vi "AT1B_Radar.vi"() -> ()   [LabVIEW 2026]
doc: "Virtuelle 4-20-mA-Kette mit eigenem Trend; keine HART- oder DTM-Verbindung. Sensor und Auswertung getrennt abgleichen. Weitere Einstellungen unterhalb der Aufnahme.\nGeometrie und liegender Zylinder sind Beispiele."
panel:
  out "Bewegungsparameter gueltig":bool=TRUE
  out "Grafikfehlercode":i32
  out "Stromverlauf [mA] - 20 ms je Punkt":dbl(graph)
  out "CSV-Fehlercode":i32
  out "Ungespeicherte Daten":bool
  out "Zeilen aufgenommen":i32
  out "Aufnahmestatus":string
  in  "Pruefstand beenden":bool
  in  "Neue CSV-Datei":path
  in  "CSV speichern":bool
  in  "Ungespeicherte Aufnahme verwerfen erlauben":bool
  in  "Neue Aufnahme":bool
  in  "Aufnahme eingeschaltet":bool
  out "Abgleichfehler (0 / 1 / 2)":dbl
  out "Signalzustand":string="Mit Ausfuehren / Strg+R starten."
  out "Messung angehalten - Anzeige historisch":bool
  out "Relais 2":bool
  out "Skalenwert":dbl=nan
  out "Auswertung linearisiert [%]":dbl=nan
  out "Auswertung [%]":dbl=nan
  out "Strom [mA]":dbl=nan
  out "Sensor linearisiert [%]":dbl=nan
  out "Sensor [%]":dbl=nan
  out "Distanz [m]":dbl=nan
  in  "Messung eingeschaltet":bool=TRUE
  in  "Auswertung uebernehmen":bool
  in  "Relais 2 Betriebsart":enum16{"Aus", "Fenster ein", "Fenster aus"}(ring)
  in  "Relais 2 Obergrenze [%]":dbl
  in  "Relais 2 Untergrenze [%]":dbl
  in  "Skalenwert bei 100 %":dbl
  in  "Skalenwert bei 0 %":dbl
  in  "Auswertung Linearisierung":enum16{"Linear", "Zylinder liegend - Beispiel"}(ring)
  in  "Auswertung Strom bei 100 % [mA]":dbl=20.0
  in  "Auswertung Strom bei 0 % [mA]":dbl=4.0
  in  "Sensorabgleich uebernehmen":bool
  in  "Sensor-Linearisierung":enum16{"Linear", "Zylinder liegend - Beispiel"}(ring)
  in  "Sensordistanz bei 100 % [m]":dbl
  in  "Sensordistanz bei 0 % [m]":dbl
  in  "Daempfung [s]":dbl
  in  "Messoffset [m] - Beispiel":dbl
  in  "Sensorhoehe ueber Boden [m] - Beispiel":dbl=1.5
  in  "Echo vorhanden":bool=TRUE
  in  "Geraete eingeschaltet":bool=TRUE
  out "Abgeschlossene Fahrten":dbl
  out "Fahrt aktiv":bool
  out "Position aktuell":dbl
  in  "Bewegung pausieren":bool
  in  "Bewegung stoppen":bool
  in  "Ablauf starten":bool
  in  "Schrittweite":dbl=0.01
  in  "Fahrtart":enum16{"Pendeln", "Schritte", "Einfachfahrt"}(ring)
  in  "Wiederholungen":dbl=1.0
  in  "Haltezeit [s]":dbl=0.5
  in  "Tempo pro Sekunde":dbl=0.05
  in  "Endposition":dbl=1.2
  in  "Startposition":dbl
  in  "Position setzen":bool
  in  "Handposition":dbl=0.3
  out "Kurzhilfe":string="Virtuelle 4-20-mA-Kette mit eigenem Trend; keine HART- oder DTM-Verbindung. Sensor und Auswertung getrennt abgleichen. Weitere Einstellungen unterhalb der Aufnahme.\nGeometrie und liegender Zylinder sind Beispiele."
  out "Pruefstand":string="AT-1B / VEGAPULS C22 und VEGAMET 391 - Fuellhoehe in m"
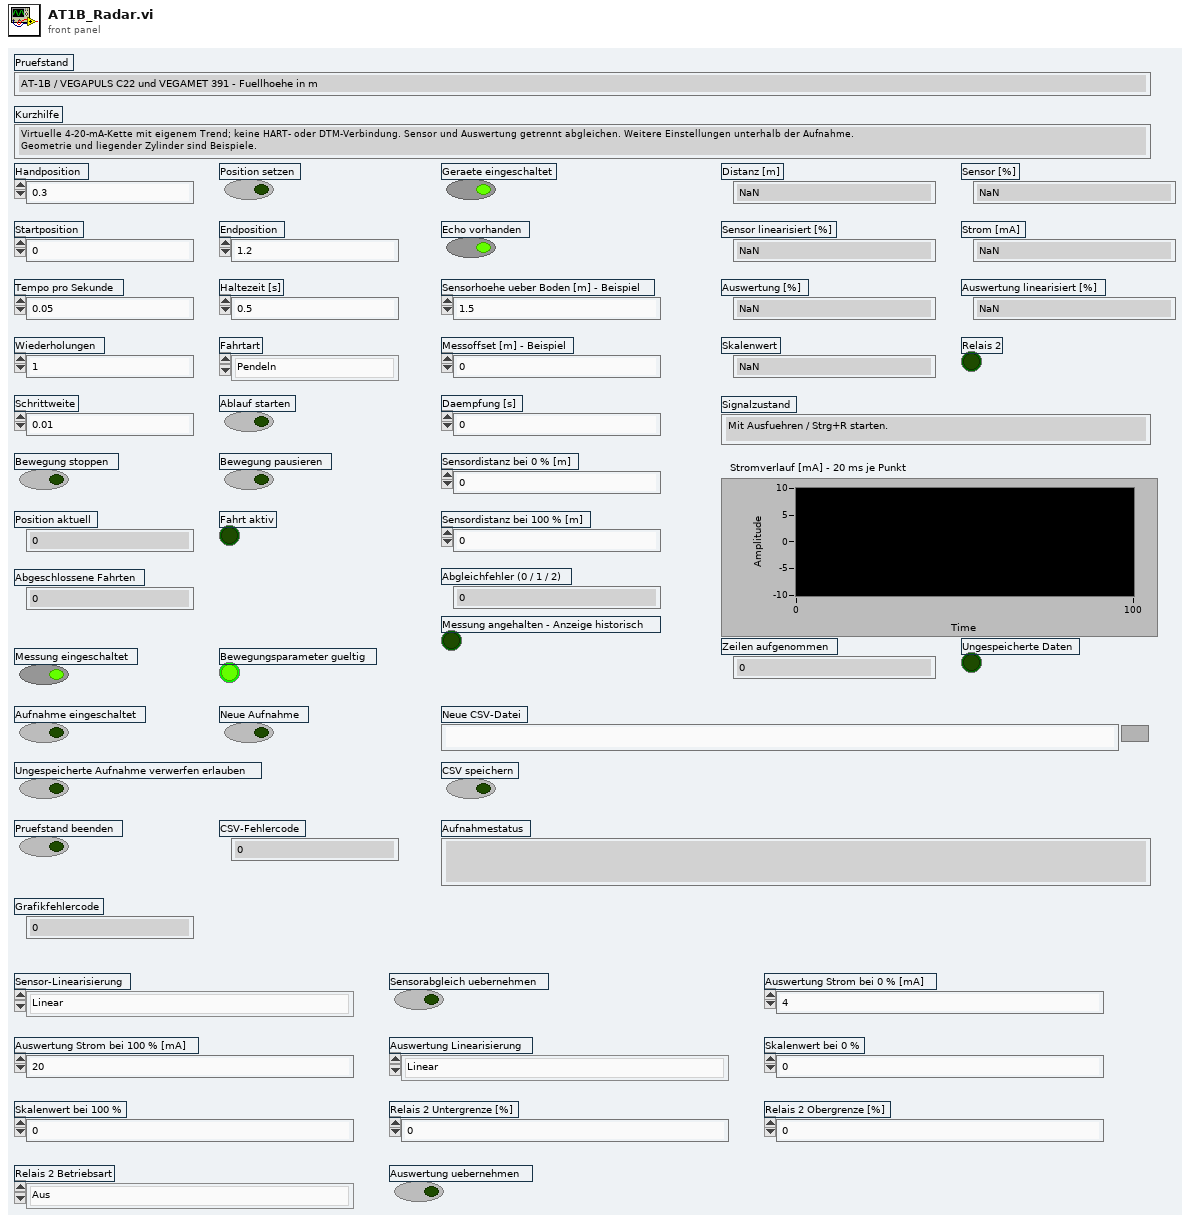
[diagram p1: front panel]
types:
  T1 = cluster{"record":bool, "clear":bool, "limit":i32, "header":string, "source":string}
diagram:
  n1 = while {
    shift-right: [w27] -> _
    shift-left: dbl[] [0.0, 0.0, 0.0, 0.0, 0.0, 0.0, 0.0, 0.0, 0.0, 0.0, 0.0, 0.0] -> [w26]
    shift-right: [w87] -> _
    shift-left: dbl[] [0.0, 0.0, 0.0, 0.0, 0.0, 0.0, 0.0, 0.0, 0.0, 0.0, 0.0, 0.0, 0.0, 0.0, 0.0, 0.0, 0.0, 0.0, 0.0, 0.0] -> [w86]
    shift-right: [w92] -> _
    shift-left: dbl[] [nan, nan, nan, nan, nan, nan, nan, nan] -> [w91]
    shift-right: [w164] -> _
    shift-left: cluster{"text":string, "count":i32} {"text"="Quelle;Zeit_s;Fuellhoehe_m;Distanz_m;Sensor_pct;Sensor_linear_pct;Strom_mA;Auswertung_pct;Auswertung_linear_pct;Skalenwert;Relais2;Qualitaet;Parameterfehler;Eingang_dt_s;Eingang_sensor_plane_above_bottom_m_example;Eingang_fill_height_m;Eingang_echo;Eingang_power;Eingang_offset_m_example;Eingang_damping_s;Eingang_sensor_distance_at_0pct_m;Eingang_sensor_distance_at_100pct_m;Eingang_sensor_linearization_0_linear_1_horizontal_cylinder;Eingang_sensor_apply_pressed;Eingang_controller_current_at_0pct_mA;Eingang_controller_current_at_100pct_mA;Eingang_controller_linearization_0_linear_1_horizontal_cylinder;Eingang_scaled_0pct;Eingang_scaled_100pct;Eingang_relay_lower_pct;Eingang_relay_upper_pct;Eingang_relay_mode_0_off_1_window_on_2_window_off;Eingang_controller_apply_pressed\r\n", "count"=0} -> [w163]
    shift-right: [w166] -> _
    shift-left: 0 -> [w165]
    shift-right: [w227] -> _
    shift-left: errorcluster {"status"=FALSE, "code"=0, "source"=""} -> [w226]
    i -> [w7]
    stop <- w243 stop-if-true
    w10 = FALSE
    (unwired) 1.0
    w9 = 0.0
    w8 = 0.02
    # "Virtueller Pruefstand - 20 ms Modellschritt"
    n2 = case shown="True" "Position setzen" {
      frame False {
      }
      frame True {
        n3 = property on="Position setzen" class="Bool. (strikt)"("Value"=FALSE) -> ()  [unwired: 2 in, 2 out]
      }
    }
    n4 = case shown="True" "Ablauf starten" {
      frame False {
      }
      frame True {
        n5 = property on="Ablauf starten" class="Bool. (strikt)"("Value"=FALSE) -> ()  [unwired: 2 in, 2 out]
      }
    }
    n6 = case shown="True" "Bewegung stoppen" {
      frame False {
      }
      frame True {
        n7 = property on="Bewegung stoppen" class="Bool. (strikt)"("Value"=FALSE) -> ()  [unwired: 2 in, 2 out]
      }
    }
    n8 = case shown="True" "Sensorabgleich uebernehmen" {
      frame False {
      }
      frame True {
        n9 = property on="Sensorabgleich uebernehmen" class="Bool. (strikt)"("Value"=FALSE) -> ()  [unwired: 2 in, 2 out]
      }
    }
    n10 = case shown="True" "Auswertung uebernehmen" {
      frame False {
      }
      frame True {
        n11 = property on="Auswertung uebernehmen" class="Bool. (strikt)"("Value"=FALSE) -> ()  [unwired: 2 in, 2 out]
      }
    }
    n12 = case shown="True" "Neue Aufnahme" {
      frame False {
      }
      frame True {
        n13 = property on="Neue Aufnahme" class="Bool. (strikt)"("Value"=FALSE) -> ()  [unwired: 2 in, 2 out]
      }
    }
    n14 = case shown="True" "CSV speichern" {
      frame False {
      }
      frame True {
        n15 = property on="CSV speichern" class="Bool. (strikt)"("Value"=FALSE) -> ()  [unwired: 2 in, 2 out]
      }
    }
    n16 = case shown="True" "Pruefstand beenden" {
      frame False {
      }
      frame True {
        n17 = property on="Pruefstand beenden" class="Bool. (strikt)"("Value"=FALSE) -> ()  [unwired: 2 in, 2 out]
      }
    }
    n18 = Wait (ms)(milliseconds to wait=u32 20) -> ()  [unwired: 1 out]
    n19 = Select(t=1.0, s="Ablauf starten", f=0.0) -> (s? t:f=w30:dbl)
    n20 = property on="Stromverlauf [mA] - 20 ms je Punkt" class="SVDiagr (strikt)"("Legend:Visible"=w10, "Palette:Visible"=w10, "Scale Legend:Visible"=w10, "Position"=cluster{"Left":i32, "Top":i32} {"Left"=735, "Top"=420}, "Plot Area:Size"=cluster{"Width":u32, "Height":u32} {"Width"=340, "Height"=110}) -> (error out=w261:errorcluster)  [unwired: 2 in, 1 out]
    n21 = Select(t=1.0, s="Bewegung pausieren", f=0.0) -> (s? t:f=w33:dbl)
    n22 = Select(t=1.0, s="Position setzen", f=0.0) -> (s? t:f=w36:dbl)
    n23 = Select(t=1.0, s="Bewegung stoppen", f=0.0) -> (s? t:f=w39:dbl)
    n24 = Select(t=1.0, s="Echo vorhanden", f=0.0) -> (s? t:f=w76:dbl)
    n25 = Select(t=1.0, s="Geraete eingeschaltet", f=0.0) -> (s? t:f=w79:dbl)
    n26 = Select(t=1.0, s="Sensorabgleich uebernehmen", f=0.0) -> (s? t:f=w82:dbl)
    n27 = Select(t=1.0, s="Auswertung uebernehmen", f=0.0) -> (s? t:f=w85:dbl)
    n28 = Not(x="Messung eingeschaltet") -> (.not. x?=→"Messung angehalten - Anzeige historisch":bool)
    n29 = And(x="Aufnahme eingeschaltet", y="Messung eingeschaltet") -> (x .and. y?=w175:bool)
    n30 = Unbundle By Name(w163) -> ("count"=w167:i32)  [unwired: 1 out]
    n31 = Equal?(x=w7, y=w9) -> ()  [unwired: 1 out]
    n32 = Quotient & Remainder(x=w7, y=5) -> (x-y*floor(x/y)=w173:i32)  [unwired: 1 out]
    n33 = Build Array(w8, "Startposition", "Endposition", "Tempo pro Sekunde", "Haltezeit [s]", "Wiederholungen", w30, w33, w36, "Handposition", "Fahrtart", "Schrittweite", w39) -> (w40:dbl[])
    n34 = Unbundle By Name(w261) -> ("code"=→"Grafikfehlercode":i32)
    n35 = Greater?(x=w167, y=w165) -> (0:w168:bool)
    n36 = Equal?(x=w173, y=w9) -> (x = y?=w174:bool)
    n37 = call "Trajektorie.vi"("StateIn"=w26, "Parameters"=w40) -> ("Values"=w41:dbl[], "StateOut"=w27:dbl[])  [unwired: 8 in]
    n38 = Not(x=w168) -> (.not. x?=w169:bool)
    n39 = And(x=w175, y=w174) -> (x .and. y?=w176:bool)
    n40 = Index Array(array=w41, index=0) -> (element=w43:dbl)
    "Position aktuell" <- w43
    n41 = Index Array(array=w41, index=3) -> (element=w45:dbl)
    n42 = Index Array(array=w41, index=4) -> (element=w47:dbl)
    n43 = Index Array(array=w41, index=1) -> (element=w51:dbl)
    n44 = Index Array(array=w41, index=2) -> (element=→"Abgeschlossene Fahrten":dbl)
    n45 = Or(x=w169, y="Ungespeicherte Aufnahme verwerfen erlauben") -> (x .or. y?=w170:bool)
    n46 = Greater?(x=w47, y=0.0) -> (0:→"Bewegungsparameter gueltig":bool)
    n47 = Greater?(x=w51, y=0.0) -> (0:→"Fahrt aktiv":bool)
    n48 = Build Array(w8, "Sensorhoehe ueber Boden [m] - Beispiel", w43, w76, w79, "Messoffset [m] - Beispiel", "Daempfung [s]", "Sensordistanz bei 0 % [m]", "Sensordistanz bei 100 % [m]", "Sensor-Linearisierung", w82, "Auswertung Strom bei 0 % [mA]", "Auswertung Strom bei 100 % [mA]", "Auswertung Linearisierung", "Skalenwert bei 0 %", "Skalenwert bei 100 %", "Relais 2 Untergrenze [%]", "Relais 2 Obergrenze [%]", "Relais 2 Betriebsart", w85) -> (w88:dbl[])
    n49 = And(x="Neue Aufnahme", y=w170) -> (x .and. y?=w171:bool)
    n50 = Not(x=w170) -> (.not. x?=w244:bool)
    n51 = call "Radar_Schritt.vi"("StateIn"=w86, "Parameters"=w88) -> ("Values"=w89:dbl[], "StateOut"=w87:dbl[])  [unwired: 8 in]
    n52 = Index Array(array=w88, index=0) -> (element=w183:dbl)
    n53 = Index Array(array=w88, index=1) -> (element=w185:dbl)
    n54 = Index Array(array=w88, index=2) -> (element=w187:dbl)
    n55 = Index Array(array=w88, index=3) -> (element=w189:dbl)
    n56 = Index Array(array=w88, index=4) -> (element=w191:dbl)
    n57 = Index Array(array=w88, index=5) -> (element=w193:dbl)
    n58 = Index Array(array=w88, index=6) -> (element=w195:dbl)
    n59 = Index Array(array=w88, index=7) -> (element=w197:dbl)
    n60 = Index Array(array=w88, index=8) -> (element=w199:dbl)
    n61 = Index Array(array=w88, index=9) -> (element=w201:dbl)
    n62 = Index Array(array=w88, index=10) -> (element=w203:dbl)
    n63 = Index Array(array=w88, index=11) -> (element=w205:dbl)
    n64 = Index Array(array=w88, index=12) -> (element=w207:dbl)
    n65 = Index Array(array=w88, index=13) -> (element=w209:dbl)
    n66 = Index Array(array=w88, index=14) -> (element=w211:dbl)
    n67 = Index Array(array=w88, index=15) -> (element=w213:dbl)
    n68 = Index Array(array=w88, index=16) -> (element=w215:dbl)
    n69 = Index Array(array=w88, index=17) -> (element=w217:dbl)
    n70 = Index Array(array=w88, index=18) -> (element=w219:dbl)
    n71 = Index Array(array=w88, index=19) -> (element=w221:dbl)
    n72 = Bundle By Name(cluster=T1 {"record"=FALSE, "clear"=FALSE, "limit"=10000, "header"="", "source"=""}, "record"=w176, "clear"=w171, "limit"=10000, "header"="Quelle;Zeit_s;Fuellhoehe_m;Distanz_m;Sensor_pct;Sensor_linear_pct;Strom_mA;Auswertung_pct;Auswertung_linear_pct;Skalenwert;Relais2;Qualitaet;Parameterfehler;Eingang_dt_s;Eingang_sensor_plane_above_bottom_m_example;Eingang_fill_height_m;Eingang_echo;Eingang_power;Eingang_offset_m_example;Eingang_damping_s;Eingang_sensor_distance_at_0pct_m;Eingang_sensor_distance_at_100pct_m;Eingang_sensor_linearization_0_linear_1_horizontal_cylinder;Eingang_sensor_apply_pressed;Eingang_controller_current_at_0pct_mA;Eingang_controller_current_at_100pct_mA;Eingang_controller_linearization_0_linear_1_horizontal_cylinder;Eingang_scaled_0pct;Eingang_scaled_100pct;Eingang_relay_lower_pct;Eingang_relay_upper_pct;Eingang_relay_mode_0_off_1_window_on_2_window_off;Eingang_controller_apply_pressed\r\n", "source"="AT1B_Radar;") -> (w181:T1)
    n73 = Select(t=errorcluster {"status"=FALSE, "code"=0, "source"=""}, s=w171, f=w226) -> (s? t:f=w232:errorcluster)
    n74 = Select(t=0, s=w171, f=w165) -> (s? t:f=w239:i32)
    n75 = And(x="Neue Aufnahme", y=w244) -> (x .and. y?=w245:bool)
    n76 = Select(t=w89, s="Messung eingeschaltet", f=w91) -> (s? t:f=w92:dbl[])
    n77 = Index Array(array=w89, index=8) -> (element=w108:dbl)
    n78 = Index Array(array=w89, index=9) -> (element=w113:dbl)
    n79 = Index Array(array=w89, index=10) -> (element=→"Abgleichfehler (0 / 1 / 2)":dbl)
    n80 = Index Array(array=w89, index=0) -> (element=w138:dbl)
    n81 = Index Array(array=w89, index=1) -> (element=w140:dbl)
    n82 = Index Array(array=w89, index=2) -> (element=w142:dbl)
    n83 = Index Array(array=w89, index=3) -> (element=w144:dbl)
    n84 = Index Array(array=w89, index=4) -> (element=w146:dbl)
    n85 = Index Array(array=w89, index=5) -> (element=w148:dbl)
    n86 = Index Array(array=w89, index=6) -> (element=w150:dbl)
    n87 = Index Array(array=w89, index=8) -> (element=w152:dbl)
    n88 = Index Array(array=w89, index=9) -> (element=w154:dbl)
    n89 = Index Array(array=w89, index=10) -> (element=w156:dbl)
    n90 = Index Array(array=w92, index=0) -> (element=→"Distanz [m]":dbl)
    n91 = Index Array(array=w92, index=1) -> (element=→"Sensor [%]":dbl)
    n92 = Index Array(array=w92, index=2) -> (element=→"Sensor linearisiert [%]":dbl)
    n93 = Index Array(array=w92, index=3) -> (element=→"Strom [mA]":dbl)
    n94 = Index Array(array=w92, index=4) -> (element=→"Auswertung [%]":dbl)
    n95 = Index Array(array=w92, index=5) -> (element=→"Auswertung linearisiert [%]":dbl)
    n96 = Index Array(array=w92, index=6) -> (element=→"Skalenwert":dbl)
    n97 = Greater?(x=w108, y=0.0) -> (0:→"Relais 2":bool)
    n98 = Equal?(x=w113, y=0.0) -> (x = y?=w116:bool)
    n99 = Equal?(x=w113, y=1.0) -> (x = y?=w120:bool)
    n100 = Equal?(x=w113, y=2.0) -> (x = y?=w124:bool)
    n101 = Equal?(x=w113, y=3.0) -> (x = y?=w128:bool)
    n102 = Equal?(x=w113, y=4.0) -> (x = y?=w132:bool)
    n103 = Build Array(w45, w43, w138, w140, w142, w144, w146, w148, w150, w152, w154, w156, w183, w185, w187, w189, w191, w193, w195, w197, w199, w201, w203, w205, w207, w209, w211, w213, w215, w217, w219, w221) -> (w222:dbl[])
    n104 = Index Array(array=w92, index=3) -> (element=→"Stromverlauf [mA] - 20 ms je Punkt":dbl)
    n105 = Select(t="Messsignal gueltig", s=w116, f="Parameter ungueltig - Eingaben pruefen.") -> (s? t:f=w118:string)
    n106 = call "Aufzeichnung_Schritt.vi"("Previous"=w163, "Row"=w222, "Settings"=w181) -> ("Full"=w223:bool, "Current"=w164:cluster{"text":string, "count":i32})  [unwired: 11 in]
    n107 = Select(t="Sensorabgleich fehlt", s=w120, f=w118) -> (s? t:f=w122:string)
    n108 = Unbundle By Name(w164) -> ("text"=w224:string, "count"=w225:i32)
    "Zeilen aufgenommen" <- w225
    n109 = Select(t="Auswertung noch nicht abgeglichen", s=w124, f=w122) -> (s? t:f=w126:string)
    n110 = Greater?(x=w225, y=0.0) -> (0:w229:bool)
    n111 = Select(t="Kein Echo", s=w128, f=w126) -> (s? t:f=w130:string)
    n112 = And(x="CSV speichern", y=w229) -> (x .and. y?=w230:bool)
    n113 = case shown="True" w230 {
      tunnel: "Neue CSV-Datei" -> [_ w264]
      tunnel: w232 -> [w263 _]
      tunnel: w224 -> [_ w265]
      tunnel: [w263 w266] -> w227
      frame False {
      }
      frame True {
        n114 = call "CSV_Speichern.vi"("Text"=w265, "Datei"=w264) -> ("error out"=w266:errorcluster)  [unwired: 13 in]
      }
    }
    n115 = Select(t="Geraete ausgeschaltet", s=w132, f=w130) -> (s? t:f=→"Signalzustand":string)
    n116 = Unbundle By Name(w227) -> ("status"=w233:bool, "code"=→"CSV-Fehlercode":i32, "source"=w235:string)
    n117 = Not(x=w233) -> (.not. x?=w236:bool)
    n118 = And(x=w230, y=w236) -> (x .and. y?=w237:bool)
    n119 = Select(t=w225, s=w237, f=w239) -> (s? t:f=w166:i32)
    n120 = Greater?(x=w225, y=w166) -> (0:w240:bool)
    "Ungespeicherte Daten" <- w240
    n121 = Not(x=w240) -> (.not. x?=w241:bool)
    n122 = Select(t="Aufnahme noch nicht gespeichert. Vor neuer Aufnahme oder Beenden CSV speichern oder Verwerfen erlauben einschalten.", s=w240, f="Bereit. Aufnahme mit neuem Dateinamen speichern.") -> (s? t:f=w251:string)
    n123 = Or(x=w241, y="Ungespeicherte Aufnahme verwerfen erlauben") -> (x .or. y?=w242:bool)
    n124 = Select(t="Aufnahme voll (10 000 Zeilen). Speichern und neue Aufnahme beginnen.", s=w223, f=w251) -> (s? t:f=w253:string)
    n125 = And(x="Pruefstand beenden", y=w242) -> (x .and. y?=w243:bool)
    n126 = Not(x=w243) -> (.not. x?=w246:bool)
    n127 = And(x="Pruefstand beenden", y=w246) -> (x .and. y?=w247:bool)
    n128 = Or(x=w245, y=w247) -> (x .or. y?=w248:bool)
    n129 = Select(t="Erst CSV speichern oder Verwerfen erlauben einschalten.", s=w248, f=w253) -> (s? t:f=w255:string)
    n130 = Select(t=w235, s=w233, f=w255) -> (s? t:f=→"Aufnahmestatus":string)
    "Pruefstand" <- "AT-1B / VEGAPULS C22 und VEGAMET 391 - Fuellhoehe in m"
    "Kurzhilfe" <- "Virtuelle 4-20-mA-Kette mit eigenem Trend; keine HART- oder DTM-Verbindung. Sensor und Auswertung getrennt abgleichen. Weitere Einstellungen unterhalb der Aufnahme.\nGeometrie und liegender Zylinder sind Beispiele."
  }
